vi "GC Collect.vi"   [LabVIEW 2026, in "ToastNotification.lvlib"]
uses:
  ToastNotification.lvlib
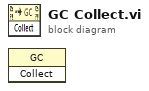
[diagram p0: block diagram]
diagram:
  n1 = invoke class="GC" method="Collect"() -> ()  [unwired: 3 in, 3 out]
